vi "Collect MCP Input Requests.vi"(8 "error in":errorcluster, 10 "input requests queue":refnum<queue>, 11 "context queue":refnum<queue>) -> (0 "error out":errorcluster, 3 "input requests":string)   [LabVIEW 2020, in "MCP Server.lvlib"]
doc: "Runs after the request was handled, and undoes Set MCP Request Context.vi: collects the questions that Ask User.vi registered in the named queue \"MCP Input Requests\" while a tool ran, takes this request's context out of the named queue \"MCP Request Context\" (which lets the next request in) and releases both queue references.\n\ninput requests is one JSON object with every registered question by its key (the inputRequests of an input_required result), or empty when no question was registered.\n\nIt runs whatever error in carries: the cleanup must happen even when handling failed. Its own queue and JSON errors are discarded, as before the split, and error in is passed through unchanged."
uses:
  MCP Server.lvlib
  <vilib>/JDP Science/JSONtext/support/Format JSON Object.vi
  <vilib>/JDP Science/JSONtext/JSONtext.lvlib
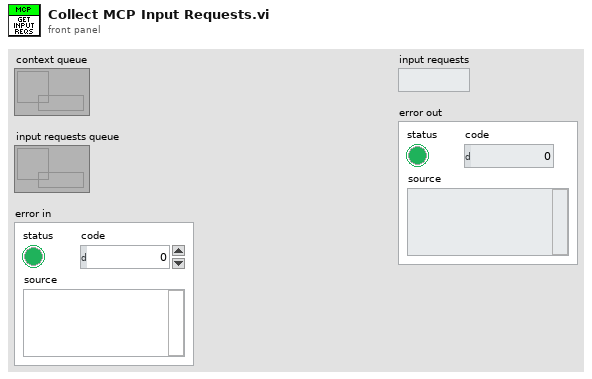
[diagram p1: front panel]
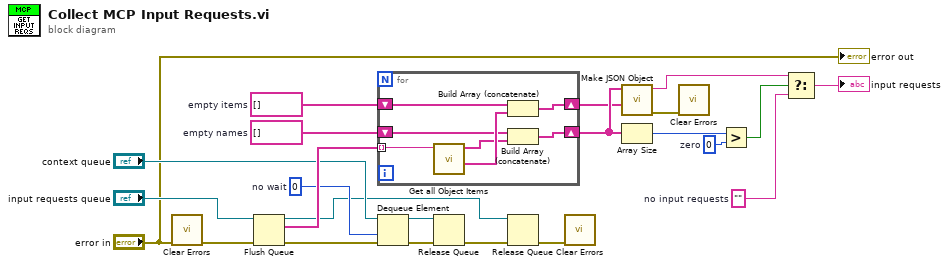
[diagram p0: block diagram]
diagram:
  w3 = ""  # no input requests
  w6 = 0  # zero
  w19 = string[] []  # empty items
  w20 = string[] []  # empty names
  w17 = 0  # no wait
  n1 = call <vilib>:"Clear Errors.vi"("error in (no error)"="error in") -> ("error out"=w22:errorcluster)  [unwired: 5 in, 1 out]
  n2 = Flush Queue(queue="input requests queue", error in (no error)=w22) -> (queue out=w13:refnum<queue>, remaining elements=w21:string[], error out=w16:errorcluster)
  n3 = for {
    tunnel: w21 -> [w30] mode=indexing
    shift-right: [w27] -> w10
    shift-left: w20 -> [w26]
    shift-right: [w25] -> w9
    shift-left: w19 -> [w24]
    n4 = call <vilib>:"Get all Object Items.vi"("JSON"=w30) -> ("<JSON>"=w29:string[], "Item Names"=w28:string[])  [unwired: 7 in, 2 out]
    n5 = Build Array (concatenate)(w24, w29) -> (w25:string[])
    n6 = Build Array (concatenate)(w26, w28) -> (w27:string[])
  }
  n7 = Dequeue Element(queue="context queue", timeout in ms (-1)=w17, error in (no error)=w16) -> (queue out=w15:refnum<queue>, error out=w14:errorcluster)  [unwired: 2 out]
  n8 = Release Queue(queue=w15, error in (no error)=w14) -> (error out=w12:errorcluster)  [unwired: 1 in, 2 out]
  n9 = Release Queue(queue=w13, error in (no error)=w12) -> (error out=w11:errorcluster)  [unwired: 1 in, 2 out]
  n10 = call <vilib>:"Clear Errors.vi"("error in (no error)"=w11) -> ()  [unwired: 5 in, 2 out]
  n11 = call <vilib>:"Make JSON Object.vi"("JSON Items"=w9, "Item Names"=w10) -> ("error out"=w8:errorcluster, "<JSON>"=w5:string)  [unwired: 8 in]
  n12 = Array Size(array=w10) -> (size(s)=w7:i32)
  n13 = call <vilib>:"Clear Errors.vi"("error in (no error)"=w8) -> ()  [unwired: 5 in, 2 out]
  n14 = Greater?(x=w7, y=w6) -> (0:w4:bool)
  n15 = Select(t=w5, s=w4, f=w3) -> (s? t:f=→"input requests":string)
  "error out" <- "error in"
